vi "insert_edge.vi"(10 "edge":refnum<class "Edge.lvclass">, 11 "graph":refnum<class "Graph.lvclass">) -> (1 "edge unchanged?":bool, 2 "edge already included?":bool, 3 "graph out":refnum<class "Graph.lvclass">)   [LabVIEW 2020, in "graph.lvlib" / "Graph.lvclass"]
uses:
  Graph.lvclass
  Edge/Edge.lvclass
  Graph.lvclass/Graph.ctl
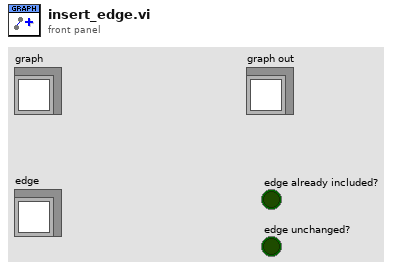
[diagram p1: front panel]
types:
  T1 = typedef "graph.lvlib/Graph.lvclass/edge-definition-cluster.ctl" = cluster{"source-id":refnum<class "ID.lvclass">, "sink-id":refnum<class "ID.lvclass">}
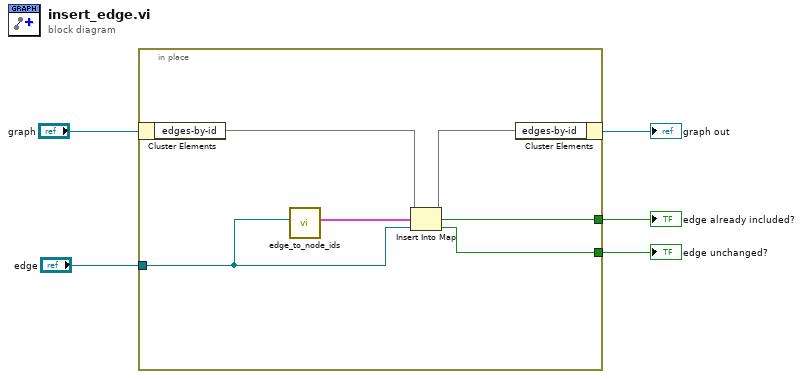
[diagram p0: block diagram]
diagram:
  n1 = in-place {
    in-place-border: [w8] -> w3
    in-place-border: "edge" -> [w7]
    in-place-border: [w9] -> w5
    n2 = in-place-cluster #1("graph") -> ("edges-by-id"=w10:map{T1, refnum<class "Edge.lvclass">})
    n3 = call "edge_to_node_ids.vi"("edge"=w7) -> ("node-ids-cluster"=w6:T1)  [unwired: 10 in]
    n4 = Insert Into Map(map in=w10, key=w6, value=w7) -> (map out=w11:map{T1, refnum<class "Edge.lvclass">}, key already included?=w8:bool, value unchanged?=w9:bool)
    n5 = in-place-cluster #1("edges-by-id"=w11) -> (→"graph out":refnum<class "Graph.lvclass">)
  }
  "edge unchanged?" <- w5
  "edge already included?" <- w3
